vi "Percent Change.vi"(10 "before":dbl=1.0, 11 "now":dbl) -> (3 "percent":dbl)   [LabVIEW 2020, in "Full Featured MCP Server.lvlib"]
doc: "Returns by how many percent a price moved from before to now, rounded to one decimal. 110 now and 100 before gives 10."
uses:
  Full Featured MCP Server.lvlib
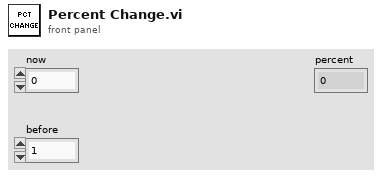
[diagram p1: front panel]
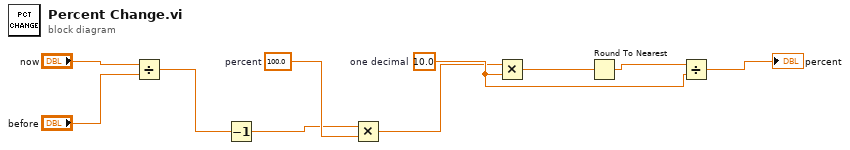
[diagram p0: block diagram]
diagram:
  w7 = 10.0  # one decimal
  w5 = 100.0  # percent
  n1 = Divide(x="now", y="before") -> (x/y=w3:dbl)
  n2 = Decrement(x=w3) -> (x-1=w4:dbl)
  n3 = Multiply(x=w4, y=w5) -> (x*y=w6:dbl)
  n4 = Multiply(x=w6, y=w7) -> (x*y=w8:dbl)
  n5 = Round To Nearest(number=w8) -> (nearest integer value=w9:dbl)
  n6 = Divide(x=w9, y=w7) -> (x/y=→"percent":dbl)
